vi "test timestamp from le bytes.vi"(8 "error in (no error)":errorcluster, 11 "TestCase in":refnum<class "Timestamp Tests.lvclass">) -> (0 "error out":errorcluster, 3 "TestCase out":refnum<class "Timestamp Tests.lvclass">)   [LabVIEW 2020, in "Timestamp Tests.lvclass"]
uses:
  Timestamp Tests.lvclass
  <vilib>/Utility/file.llb/Application Directory.vi
  <vilib>/Utility/libraryn.llb/Check if File or Folder Exists.vi
  <vilib>/addons/_JKI Toolkits/VI Tester/TestCase.llb/TestCase.lvclass
  C:/Program Files/National Instruments/LabVIEW 2024/vi.lib/addons/_JKI Toolkits/VI Tester/TestCase.llb/TestCase.lvclass
panel:
  out "data string 2":string
  out "data string":string
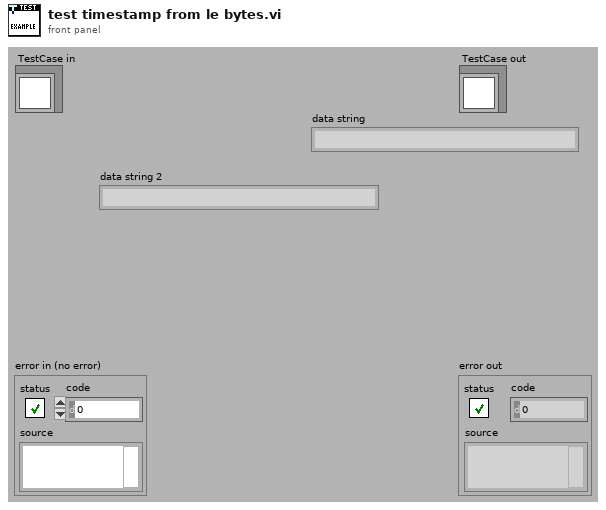
[diagram p1: front panel]
types:
  T1 = enum16{"big-endian, network order", "native, host order", "little-endian"}
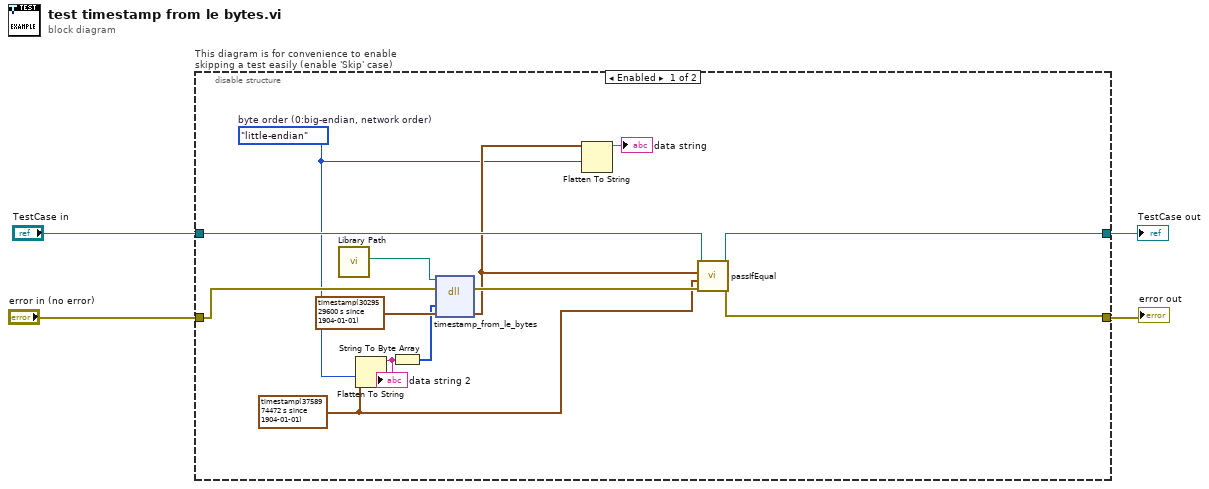
[diagram p0: block diagram]
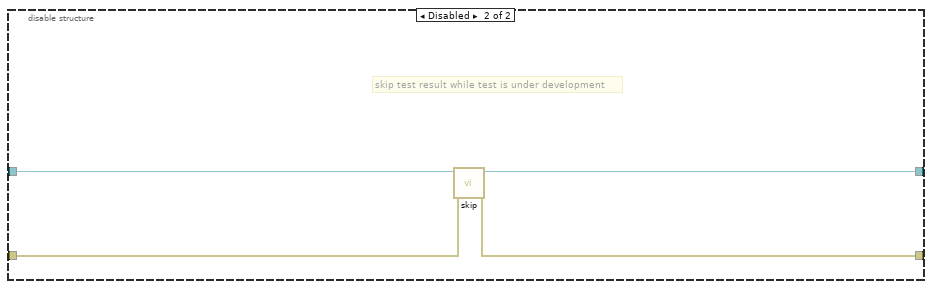
[diagram p2: hidden frame]
diagram:
  n1 = disable-structure "This diagram is for convenience to enable skipping a test easily (enable 'Skip' case)" shown="Enabled" {
    disable-tunnel: "TestCase in" -> [w17 w21]
    disable-tunnel: [w16 w19] -> w1
    disable-tunnel: [w15 w20] -> w3
    disable-tunnel: "error in (no error)" -> [w14 w18]
    frame Enabled {
      w5 = T1."little-endian"  # byte order (0:big-endian, network order)
      w11 = timestamp(3758974472.02441 s since 1904-01-01) ("Time Stamp")
      n2 = call "Library Path.vi"() -> ("Library Path"=w8:path)  [unwired: 11 in]
      n3 = Flatten To String(anything=w11, byte order (0:big-endian, network order)=w5) -> (data string=w10:string)  [unwired: 2 in, 2 out]
      "data string 2" <- w10
      n4 = String To Byte Array(string=w10) -> (unsigned byte array=w9:u8[])
      n5 = dll-call lib="C:/Users/JamesMcNally/Documents/RustInterop/Rust-LabVIEW-Interop/target/debug/labview_test_library.dll" fn="timestamp_from_le_bytes"(path in=w8, error in=w14, "bytes"=w9, "timestamp"=timestamp(3029529600 s since 1904-01-01) ("Time Stamp")) -> (error out=w13:errorcluster, "timestamp"=w6:timestamp)  [unwired: 3 in, 1 out]
      n6 = Flatten To String(anything=w6, byte order (0:big-endian, network order)=w5) -> (data string=→"data string":string)  [unwired: 2 in, 2 out]
      n7 = call-dynamic "passIfEqual.vi"("error in (no error)"=w13, "y"=w11, "x"=w6, "TestCase in"=w17) -> ("error out"=w15:errorcluster, "TestCase out"=w16:refnum<class "Timestamp Tests.lvclass">)  [unwired: 6 in]
    }
    frame Disabled {
      # "skip test result while test is under development"
      n8 = call <vilib>:"skip.vi"("error in (no error)"=w18, "TestCase in"=w21) -> ("error out"=w20:errorcluster, "TestCase out"=w19:refnum<class "Timestamp Tests.lvclass">)  [unwired: 8 in]
    }
  }
  "error out" <- w3
  "TestCase out" <- w1
